vi "Echo_Send_Report.vi"(6 "frame":T3 {"id" format="%.0x"}, 7 "context":T5 {"ack hi" format="%.0x"; "ack lo" format="%.0x"; "test hi" format="%.0x"; "test lo" format="%.0x"}, 8 "error in (no error)":errorcluster, 9 "counters in":T1, 10 "time store in":T2) -> (0 "error out":errorcluster, 1 "counters out":T1, 2 "time store out":T2)   [LabVIEW 2021]
doc: "echo, Ack case: looks up the times at key. If an echo was stored (t_rx2_dev > 0): 36-byte Echo_Report (big-endian) by UDP to lv addr:report port, entry cleared, TX acks matched + 1. Else unmatched acks + 1. time store changes in place."
uses:
  common/Typedefs/Echo_Report.ctl
  common/CANsub_Common.lvlib
  Echo_Time_Store.ctl
  Echo_Counters.ctl
  Echo_Context.ctl
  Echo_Frame_Kind.ctl
  Echo_Frame.ctl
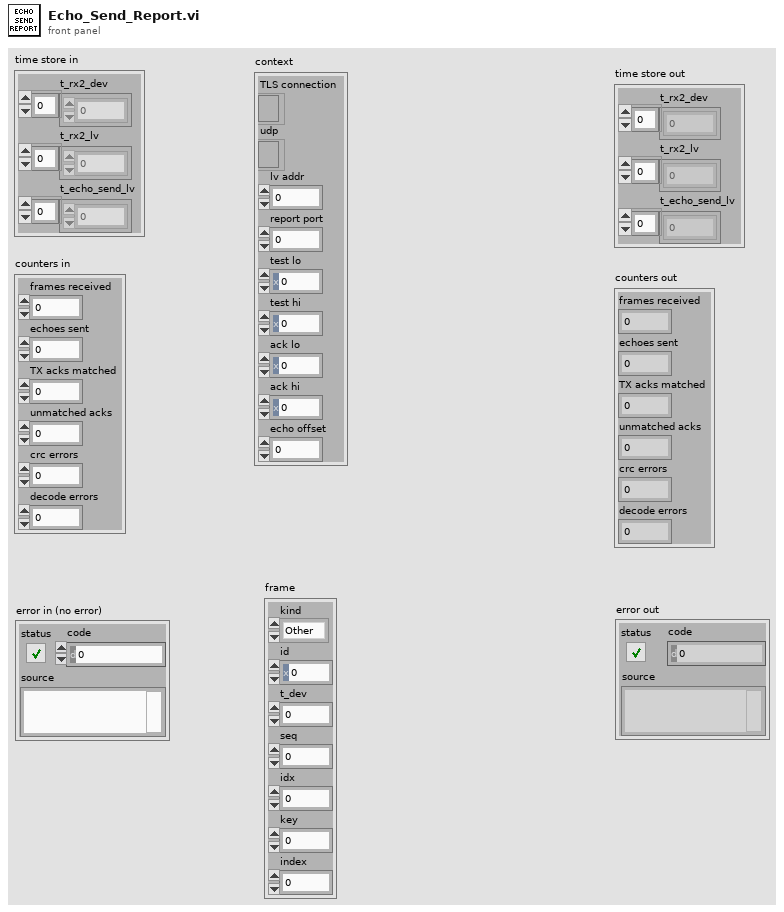
[diagram p1: front panel]
types:
  T1 = typedef "Echo_Counters.ctl" = cluster{"frames received":u32, "echoes sent":u32, "TX acks matched":u32, "unmatched acks":u32, "crc errors":u32, "decode errors":i32}
  T2 = typedef "Echo_Time_Store.ctl" = cluster{"t_rx2_dev":dbl[], "t_rx2_lv":dbl[], "t_echo_send_lv":dbl[]}
  T3 = typedef "Echo_Frame.ctl" = cluster{"kind":T4, "id":u32, "t_dev":dbl, "seq":u16, "idx":u8, "key":i32, "index":i32}
  T4 = typedef "Echo_Frame_Kind.ctl" = enum16{"Other", "Test", "Ack"}
  T5 = typedef "Echo_Context.ctl" = cluster{"TLS connection":refnum<k5>, "udp":refnum<k16>, "lv addr":u32, "report port":u16, "test lo":u32, "test hi":u32, "ack lo":u32, "ack hi":u32, "echo offset":i32}
  T6 = enum16{"big-endian, network order", "native, host order", "little-endian"}
  T7 = typedef "CANsub_Common.lvlib/Echo_Report.ctl" = cluster{"seq":u16, "idx":u8, "pad":u8, "t_rx2_dev":dbl, "t_echo_txack2_dev":dbl, "t_rx2_lv":dbl, "t_echo_send_lv":dbl}
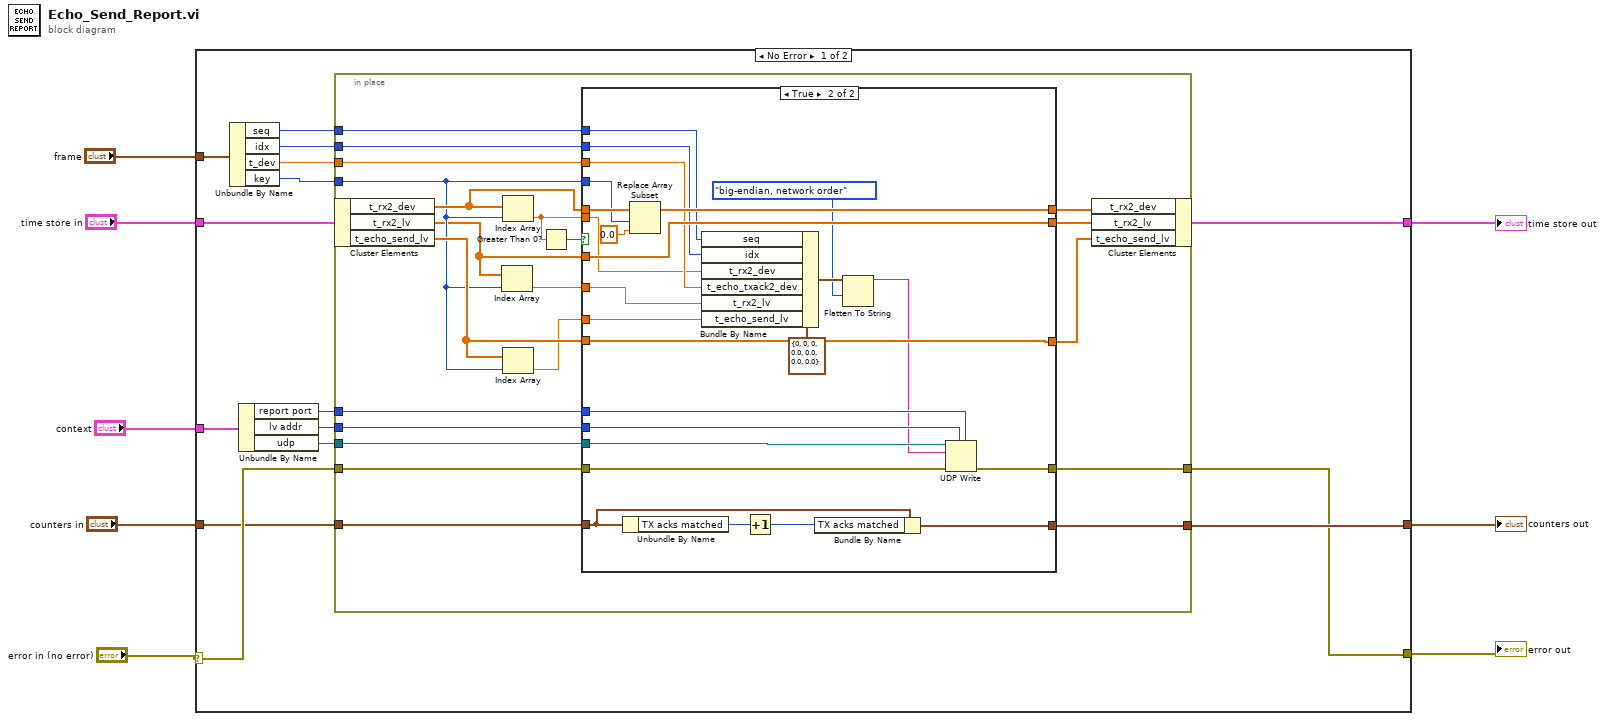
[diagram p0: block diagram]
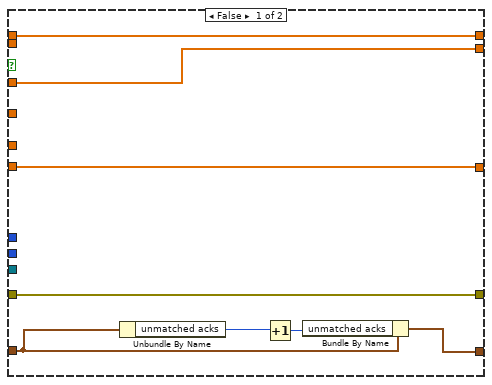
[diagram p2: hidden frame]
diagram:
  n1 = case shown="No Error" "error in (no error)" {
    selector: "error in (no error)" -> [w20 w80]
    tunnel: [w15 w80] -> w7
    tunnel: [w17 w79] -> w6
    tunnel: "time store in" -> [w23 w79]
    tunnel: [w16 w78] -> w4
    tunnel: "counters in" -> [w19 w78]
    tunnel: "context" -> [w22 _]
    tunnel: "frame" -> [w21 _]
    frame No Error {
      n2 = Unbundle By Name(w21) -> ("seq"=w14:u16, "idx"=w13:u8, "t_dev"=w12:dbl, "key"=w18:i32)
      n3 = Unbundle By Name(w22) -> ("report port"=w11:u16, "lv addr"=w10:u32, "udp"=w9:refnum<k16>)
      n4 = in-place {
        in-place-border: w20 -> [w42]
        in-place-border: w19 -> [w36]
        in-place-border: w18 -> [w34]
        in-place-border: [w43] -> w15
        in-place-border: [w35] -> w16
        in-place-border: w14 -> [w32]
        in-place-border: w13 -> [w31]
        in-place-border: w12 -> [w30]
        in-place-border: w11 -> [w26]
        in-place-border: w10 -> [w25]
        in-place-border: w9 -> [w24]
        n5 = in-place-cluster #1(w23) -> ("t_rx2_dev"=w37:dbl[], "t_rx2_lv"=w33:dbl[], "t_echo_send_lv"=w40:dbl[])
        n6 = Index Array(array=w33, index=w34) -> (element=w28:dbl)
        n7 = Index Array(array=w37, index=w34) -> (element=w29:dbl)
        n8 = Index Array(array=w40, index=w34) -> (element=w27:dbl)
        n9 = Greater Than 0?(x=w29) -> (x > 0?=w44:bool)
        n10 = case shown="True" w44 {
          tunnel: [w52 w60] -> w43
          tunnel: w42 -> [w52 w61]
          tunnel: [w51 w72] -> w41
          tunnel: w40 -> [w51 w72]
          tunnel: [w50 w73] -> w39
          tunnel: w33 -> [w50 w73]
          tunnel: [w49 w74] -> w38
          tunnel: w37 -> [w49 w77]
          tunnel: w36 -> [w48 w55]
          tunnel: [w45 w53] -> w35
          tunnel: w34 -> [_ w76]
          tunnel: w32 -> [_ w70]
          tunnel: w31 -> [_ w69]
          tunnel: w30 -> [_ w68]
          tunnel: w29 -> [_ w67]
          tunnel: w28 -> [_ w66]
          tunnel: w27 -> [_ w65]
          tunnel: w26 -> [_ w59]
          tunnel: w25 -> [_ w62]
          tunnel: w24 -> [_ w58]
          frame False {
            n11 = Unbundle By Name(w48) -> ("unmatched acks"=w47:u32)
            n12 = Increment(x=w47) -> (x+1=w46:u32)
            n13 = Bundle By Name(cluster=w48, "unmatched acks"=w46) -> (w45:T1)
          }
          frame True {
            n14 = Unbundle By Name(w55) -> ("TX acks matched"=w56:u32)
            n15 = Replace Array Subset(array=w77, new element=0.0 ("new element/subarray"), index=w76) -> (w74:dbl[])
            n16 = Bundle By Name(cluster=T7 {"seq"=0, "idx"=0, "pad"=0, "t_rx2_dev"=0.0, "t_echo_txack2_dev"=0.0, "t_rx2_lv"=0.0, "t_echo_send_lv"=0.0} ("Echo_Report"), "seq"=w70, "idx"=w69, "t_rx2_dev"=w67, "t_echo_txack2_dev"=w68, "t_rx2_lv"=w66, "t_echo_send_lv"=w65) -> (w64:T7)
            n17 = Increment(x=w56) -> (x+1=w54:u32)
            n18 = Bundle By Name(cluster=w55, "TX acks matched"=w54) -> (w53:T1)
            n19 = Flatten To String(anything=w64, byte order (0:big-endian, network order)=T6."big-endian, network order") -> (data string=w57:string)  [unwired: 2 in, 2 out]
            n20 = UDP Write(address=w62, port or service name=w59, connection ID=w58, data in=w57, 8:w61) -> (error out=w60:errorcluster)  [unwired: 1 in, 1 out]
          }
        }
        n21 = in-place-cluster #1("t_rx2_dev"=w38, "t_rx2_lv"=w39, "t_echo_send_lv"=w41) -> (w17:T2)
      }
    }
    frame Error {
    }
  }
  "error out" <- w7
  "time store out" <- w6
  "counters out" <- w4
